vi "Write Waiting Time(ms).vi"(8 "error in (no error)":errorcluster, 10 "Waiting Time(ms)":u32, 11 "NR in":refnum<class "NR.lvclass">) -> (0 "error out":errorcluster, 3 "NR out":refnum<class "NR.lvclass">)   [LabVIEW 2023, in "ANRITSU Call Box.lvlib" / "NR.lvclass"]
uses:
  NR.lvclass
  NR.lvclass/NR.ctl
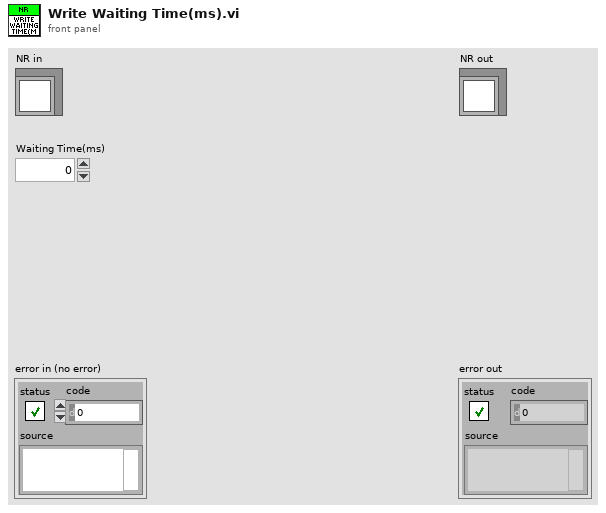
[diagram p1: front panel]
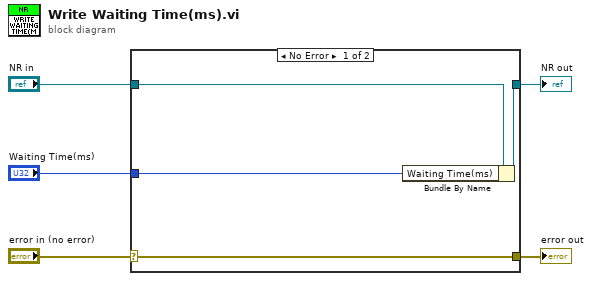
[diagram p0: block diagram]
diagram:
  n1 = case shown="No Error" "error in (no error)" {
    selector: "error in (no error)" -> [w9 w10]
    tunnel: [w9 w10] -> w4
    tunnel: [w7 w11] -> w2
    tunnel: "NR in" -> [w8 w11]
    tunnel: "Waiting Time(ms)" -> [w6 _]
    frame No Error {
      n2 = Bundle By Name(cluster=w8, "Waiting Time(ms)"=w6) -> (w7:refnum<class "NR.lvclass">)
    }
    frame Error {
    }
  }
  "error out" <- w4
  "NR out" <- w2
